vi "isPrivateURL.vi"(11 "URL":string) -> (2 "private?":bool, 3 "URL (dup)":string)   [LabVIEW 2017, in "TagDB.lvlib"]
doc: "[Covers: REQ_TAGDB_NAME]\n[Covers: REQ_TAGDB_TEMPNAME]"
uses:
  TagDB.lvlib
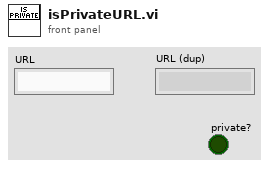
[diagram p1: front panel]
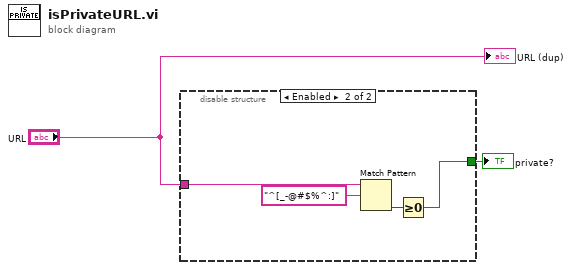
[diagram p0: block diagram]
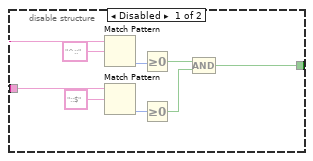
[diagram p2: hidden frame]
diagram:
  n1 = disable-structure shown="Enabled" {
    disable-tunnel: [w10 w11] -> w2
    disable-tunnel: "URL" -> [w3 w12]
    frame Disabled {
      n2 = Match Pattern(string=w3, regular expression="^::") -> (offset past match=w6:i32)  [unwired: 1 in, 3 out]
      n3 = Match Pattern(string=w3, regular expression="::$") -> (offset past match=w7:i32)  [unwired: 1 in, 3 out]
      n4 = Greater Or Equal To 0?(x=w6) -> (x >= 0?=w8:bool)
      n5 = Greater Or Equal To 0?(x=w7) -> (x >= 0?=w9:bool)
      n6 = Compound Arithmetic op=AND(w8, w9) -> (w10:bool)
    }
    frame Enabled {
      n7 = Match Pattern(string=w12, regular expression="^[_-@#$%^:]") -> (offset past match=w14:i32)  [unwired: 1 in, 3 out]
      n8 = Greater Or Equal To 0?(x=w14) -> (x >= 0?=w11:bool)
    }
  }
  "private?" <- w2
  "URL (dup)" <- "URL"
